vi "RunCore.vi"(8 "error in":errorcluster) -> (0 "error out":errorcluster)   [LabVIEW 2016, in "Drona.lvlib"]
doc: "Gets all the test paths in a packed project library and runs the test VIs"
uses:
  Drona.lvlib
  Stimulus/VI/RunVI.vi
  <vilib>/Utility/LVLibp/NI_PackedLibraryUtility.lvlib
  <vilib>/addons/_JKI Toolkits/Caraya/classes/Test/Test.lvclass
  Stimulus/VI/VI.lvlib
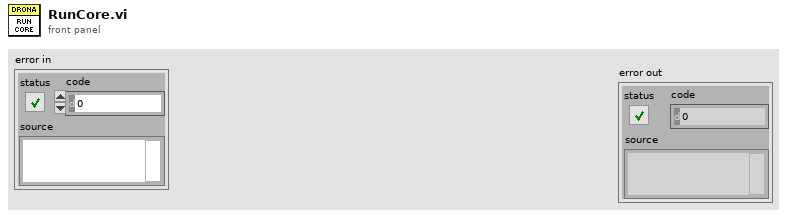
[diagram p1: front panel]
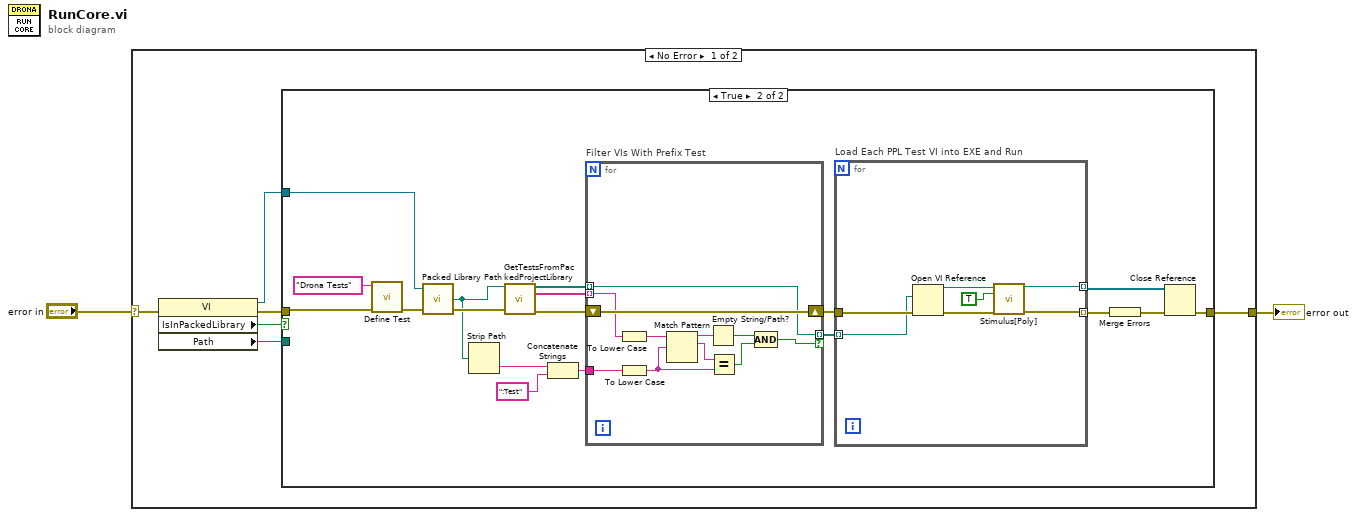
[diagram p0: block diagram]
diagram:
  n1 = case shown="No Error" "error in" {
    selector: "error in" -> [w8 w46]
    tunnel: [w4 w46] -> w2
    frame No Error {
      n2 = property class="VI"(error in=w8) -> (reference out=w5:refnum<vi>, error out=w7:errorcluster, "IsInPackedLibrary"=w6:bool, "Path"=w3:path)  [unwired: 1 in]
      n3 = case shown="True" w6 {
        tunnel: w7 -> [w9 w25]
        tunnel: w5 -> [_ w24]
        tunnel: [w9 w22] -> w4
        tunnel: w3 -> [_ _]
        frame False {
        }
        frame True {
          n4 = call <vilib>:"Define Test.vi"("error in (no error)"=w25, "Label (VI Title)"="Drona Tests") -> ("error out"=w21:errorcluster)  [unwired: 8 in, 1 out]
          n5 = call <vilib>:"Packed Library Path.vi"("error in (no error)"=w21, "vi reference"=w24) -> ("error out"=w23:errorcluster, "packed library path"=w11:path)  [unwired: 1 in, 1 out]
          n6 = Strip Path(path=w11) -> (name=w13:string)  [unwired: 1 out]
          n7 = call "GetTestsFromPackedProjectLibrary.vi"("Packed Project Library Path"=w11, "error in (no error)"=w23) -> ("Tests"=w18:path[], "Qualified Names"=w14:string[], "error out"=w17:errorcluster)  [unwired: 11 in]
          n8 = Concatenate Strings(w13, ":Test" ("string")) -> (w10:string)
          n9 = for "Filter VIs With Prefix Test" {
            tunnel: w18 -> [w37] mode=indexing
            tunnel: [w37] -> w16 mode=indexing if=w30
            shift-right: [w38] -> w15
            shift-left: w17 -> [w38]
            tunnel: w14 -> [w31] mode=indexing
            tunnel: w10 -> [w32]
            n10 = To Lower Case(string=w31) -> (all lower case string=w28:string)
            n11 = To Lower Case(string=w32) -> (all lower case string=w29:string)
            n12 = Match Pattern(string=w28, regular expression=w29) -> (before substring=w36:string, match substring=w35:string)  [unwired: 1 in, 2 out]
            n13 = Empty String/Path?(string/path=w36) -> (empty?=w34:bool)
            n14 = Equal?(x=w35, y=w29) -> (x = y?=w33:bool)
            n15 = Compound Arithmetic op=AND(w34, w33) -> (w30:bool)
          }
          n16 = for "Load Each PPL Test VI into EXE and Run" {
            tunnel: w16 -> [w40] mode=indexing
            tunnel: [w43] -> w26 mode=indexing
            tunnel: w15 -> [w42]
            tunnel: [w45] -> w27 mode=indexing
            n17 = Open VI Reference(vi path=w40, error in (no error)=w42) -> (vi reference=w39:refnum<vi>, error out=w41:errorcluster)  [unwired: 4 in]
            n18 = call-poly "Stimulus[Poly].vi"("VI Reference In"=w39, "Wait Until Done (F)"=TRUE, "error in"=w41) -> ("VI Reference Out"=w43:refnum<vi>, "error out"=w45:errorcluster)  [unwired: 11 in]
          }
          n19 = Merge Errors(w27) -> (w19:errorcluster)
          n20 = Close Reference(reference=w26, error in (no error)=w19) -> (error out=w22:errorcluster)
        }
      }
    }
    frame Error {
    }
  }
  "error out" <- w2
